vi "Set Lock.vi"(8 "error in (no error)":errorcluster, 10 "LockName":string, 11 "Tag in":refnum<class "Tag.lvclass">) -> (0 "error out":errorcluster, 3 "Tag out":refnum<class "Tag.lvclass">)   [LabVIEW 2020, in "Tag Engine Core.lvlib" / "Tag.lvclass"]
doc: "Adds a lock named LockName to the Tag and sets Locked to TRUE. A Tag can hold several named locks, and stays locked until all of them are released."
uses:
  Tag.lvclass
  Tag.lvclass/Tag.ctl
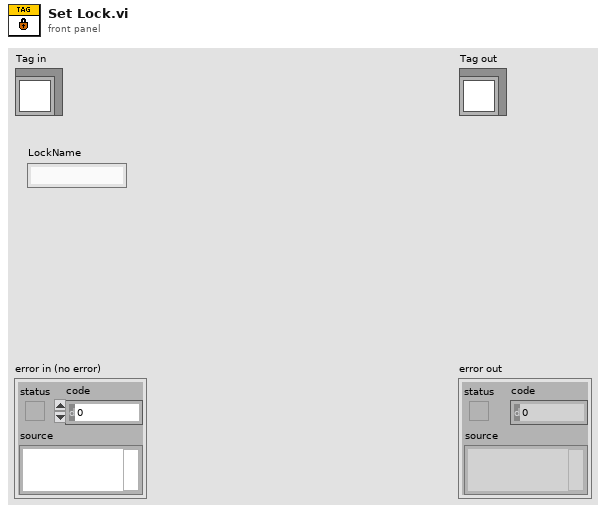
[diagram p1: front panel]
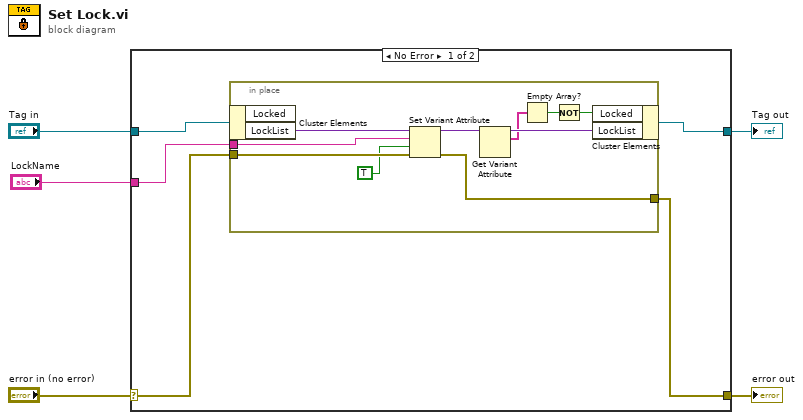
[diagram p0: block diagram]
diagram:
  n1 = case shown="No Error" "error in (no error)" {
    selector: "error in (no error)" -> [w8 w22]
    tunnel: [w7 w22] -> w4
    tunnel: [w9 w21] -> w2
    tunnel: "Tag in" -> [w10 w21]
    tunnel: "LockName" -> [w6 _]
    frame No Error {
      n2 = in-place {
        in-place-border: w8 -> [w19]
        in-place-border: [w18] -> w7
        in-place-border: w6 -> [w17]
        n3 = in-place-cluster #1(w10) -> ("LockList"=w20:variant)  [unwired: 1 out]
        n4 = Set Variant Attribute(Variant=w20, name=w17, value=TRUE, error in=w19) -> (Variant out=w15:variant, error out=w18:errorcluster)  [unwired: 1 out]
        n5 = Get Variant Attribute(Variant=w15) -> (duplicate Variant=w14:variant, names=w13:string[])  [unwired: 3 in, 2 out]
        n6 = Empty Array?(array=w13) -> (empty?=w12:bool)
        n7 = Not(x=w12) -> (.not. x?=w11:bool)
        n8 = in-place-cluster #1("Locked"=w11, "LockList"=w14) -> (w9:refnum<class "Tag.lvclass">)
      }
    }
    frame Error {
    }
  }
  "error out" <- w4
  "Tag out" <- w2
